vi "Update Displays.vi"(8 "error in":errorcluster, 10 "Status":string, 11 "Sequence Executor in":refnum<class "Sequence Executor.lvclass">) -> (0 "error out":errorcluster, 3 "Sequence Executor out":refnum<class "Sequence Executor.lvclass">)   [LabVIEW 2026, in "Sequence Executor.lvclass"]
doc: "Helper. Writes Status (input), the current step number (Step Index + 1), the step table (Build Step Table of Sequence and Results) and the Overall Verdict through the stored display references. Display errors (invalid or null references) are cleared and never returned. The object is not changed."
uses:
  Sequence Executor.lvclass
  Sequence Executor.lvclass/Sequence Executor.ctl
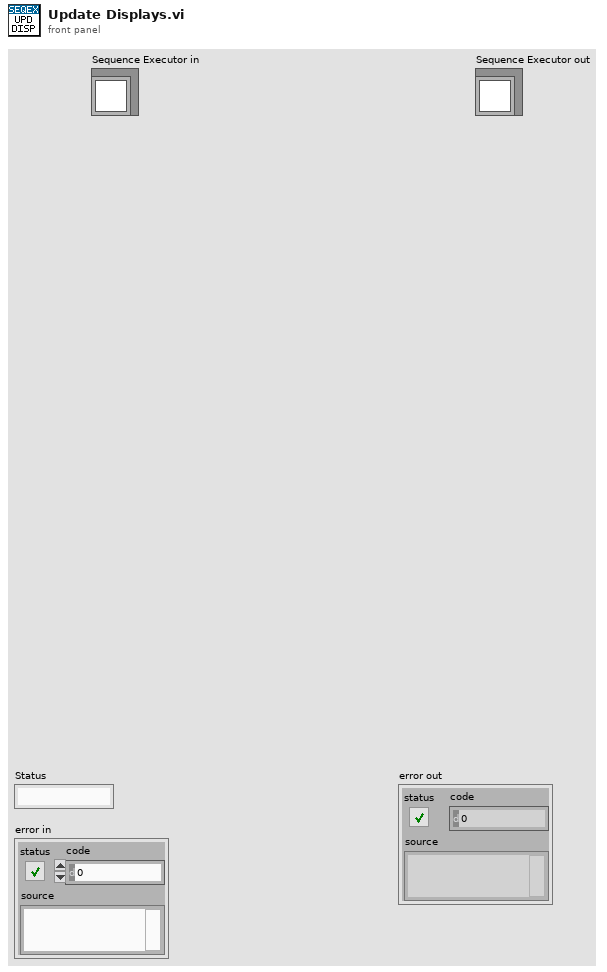
[diagram p1: front panel]
types:
  T1 = typedef "Sequence File.ctl" = cluster{"sequence_id":string, "description":string, "total_steps":i32, "steps":T2[]}
  T2 = typedef "Step Config.ctl" = cluster{"step_no":i32, "step_name":string, "command_type":string, "pressure_sp_bar":dbl, "flow_sp_lpm":dbl, "displacement_sp_mm":dbl, "monitored_io":string, "tolerance_bar":dbl, "dwell_time_ms":i32, "timeout_ms":i32, "expected_result":string}
  T3 = typedef "Step Result.ctl" = cluster{"step_no":i32, "step_name":string, "result":string, "reason":string, "measured":dbl, "target":dbl, "duration_ms":dbl}
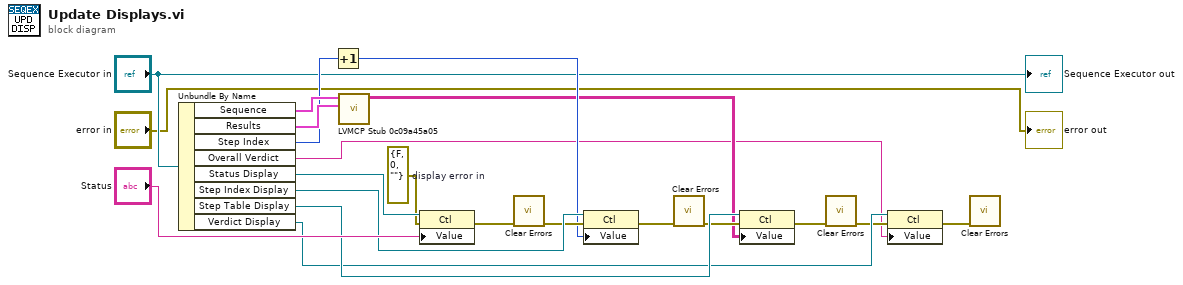
[diagram p0: block diagram]
diagram:
  w17 = errorcluster {"status"=FALSE, "code"=0, "source"=""}  # display error in
  n1 = Unbundle By Name("Sequence Executor in") -> ("Sequence"=w21:T1, "Results"=w20:T3[], "Step Index"=w19:i32, "Overall Verdict"=w4:string, "Status Display"=w18:refnum<vi>, "Step Index Display"=w14:refnum<vi>, "Step Table Display"=w10:refnum<vi>, "Verdict Display"=w6:refnum<vi>)
  n2 = Increment(x=w19) -> (x+1=w12:i32)
  n3 = call <userlib>:"LVMCP Stub 0c09a45a05.vi"("Step Results"=w20, "Sequence File"=w21) -> ("Step Table"=w8:string[][])  [unwired: 9 in]
  n4 = property class="Ctl"(reference=w18, error in=w17, "Value"="Status") -> (error out=w15:errorcluster)  [unwired: 1 out]
  n5 = call <vilib>:"Clear Errors.vi"("error in (no error)"=w15) -> ("error out"=w13:errorcluster)  [unwired: 5 in, 1 out]
  n6 = property class="Ctl"(reference=w14, error in=w13, "Value"=w12) -> (error out=w11:errorcluster)  [unwired: 1 out]
  n7 = call <vilib>:"Clear Errors.vi"("error in (no error)"=w11) -> ("error out"=w9:errorcluster)  [unwired: 5 in, 1 out]
  n8 = property class="Ctl"(reference=w10, error in=w9, "Value"=w8) -> (error out=w7:errorcluster)  [unwired: 1 out]
  n9 = call <vilib>:"Clear Errors.vi"("error in (no error)"=w7) -> ("error out"=w5:errorcluster)  [unwired: 5 in, 1 out]
  n10 = property class="Ctl"(reference=w6, error in=w5, "Value"=w4) -> (error out=w3:errorcluster)  [unwired: 1 out]
  n11 = call <vilib>:"Clear Errors.vi"("error in (no error)"=w3) -> ()  [unwired: 5 in, 2 out]
  "Sequence Executor out" <- "Sequence Executor in"
  "error out" <- "error in"
